vi "FuncVI-ss.vi"(5 "InstanceRef":T2, 9 "arg list":T1[](array[typedef]) {"num" format="%.2f"}) -> (0 "error out":bool, 3 "result":T1 {"num" format="%.2f"})   [LabVIEW 2021]
doc: "::: CalcExpress Toolkit :::\nCopyright (c) 2000-2026 Konstantin Shifershteyn. All rights reserved."
uses:
  cetypes.llb/CalcExpress Function Argument Info.ctl
  cetypes.llb/CalcExpress Instance RefNum.ctl
panel:
  in  "max arg num":i32=4
  in  "min arg num":i32=1
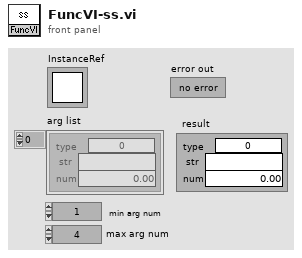
[diagram p1: front panel]
types:
  T1 = typedef "CalcExpress Function Argument Info.ctl" = cluster{"type":u32, "str":string, "num":dbl}
  T2 = typedef "CalcExpress Instance RefNum.ctl" = refnum<k1>
  T3 = cluster{"index":i32, "any type":i32, "default num":dbl, "default str":string}
  T4 = cluster{"index":i32, "data type":enum32{"String", "DBL Number", "identifier", "1D Array of DBL", "2D Array of DBL", "CDB Number", "1D Array of CDB", "2D Array of CDB", "1D Array of String", "2D Array of String", "Unknown data type"}, "default num":dbl, "default str":string}[]
  T5 = cluster{"data type":enum32{"String", "DBL Number", "identifier", "1D Array of DBL", "2D Array of DBL", "CDB Number", "1D Array of CDB", "2D Array of CDB", "1D Array of String", "2D Array of String", "Unknown data type"}, "str":string, "num":dbl}
  T6 = cluster{"index":i32, "data type":u32, "default num":dbl, "default str":string}[]
  T7 = enum32{"String", "DBL Number", "identifier", "1D Array of DBL", "2D Array of DBL", "CDB Number", "1D Array of CDB", "2D Array of CDB", "1D Array of String", "2D Array of String", "Unknown data type"}
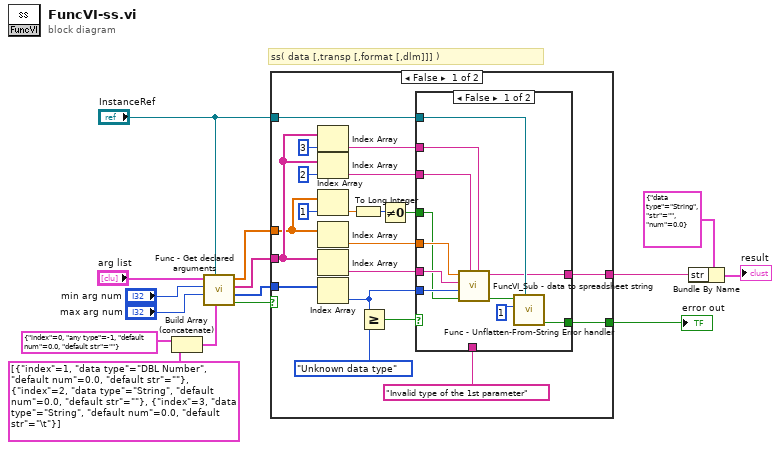
[diagram p0: block diagram]
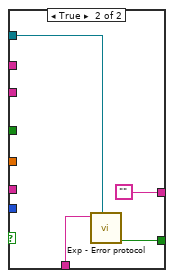
[diagram p2: hidden frame]
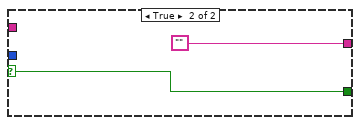
[diagram p3: hidden frame]
diagram:
  # "ss( data [,transp [,format [,dlm]]] )"
  n1 = Build Array (concatenate)(T3 {"index"=0, "any type"=-1, "default num"=0.0, "default str"=""} ("arg descriptor"), T4 [{"index"=1, "data type"=enum."DBL Number", "default num"=0.0, "default str"=""}, {"index"=2, "data type"=enum."String", "default num"=0.0, "default str"=""}, {"index"=3, "data type"=enum."String", "default num"=0.0, "default str"="\t"}] ("args descriptors")) -> (w10:T6)
  n2 = call "Func - Get declared arguments.vi"("arg descriptors"=w10, "InstanceRef"="InstanceRef", "max arg num"="max arg num", "min arg num"="min arg num", "arg list"="arg list") -> ("error out"=w9:bool, "type list"=w8:u32[], "str list"=w7:string[], "num list"=w6:dbl[])  [unwired: 3 in]
  n3 = case shown="False" w9 {
    selector: w9 -> [_ w52]
    tunnel: w8 -> [w33 _]
    tunnel: w7 -> [w32 _]
    tunnel: w6 -> [w19 _]
    tunnel: [w24 w52] -> w5
    tunnel: "InstanceRef" -> [w22 _]
    tunnel: [w21 ""] -> w3
    frame False {
      n4 = Index Array(array=w32, index=3) -> (element=w25:string)
      n5 = Index Array(array=w32, index=2) -> (element=w26:string)
      n6 = Index Array(array=w19, index=1) -> (element=w18:dbl)
      n7 = Index Array(array=w19) -> (element=w27:dbl)  [unwired: 1 in]
      n8 = Index Array(array=w32) -> (element=w28:string)  [unwired: 1 in]
      n9 = Index Array(array=w33) -> (element=w29:u32)  [unwired: 1 in]
      n10 = To Long Integer(number=w18) -> (32bit integer=w17:i32)
      n11 = Greater Or Equal?(x=w29, y=T7."Unknown data type" ("data type")) -> (x >= y?=w30:bool)
      n12 = Not Equal To 0?(x=w17) -> (x != 0?=w16:bool)
      n13 = case shown="False" w30 {
        tunnel: w29 -> [w46 _]
        tunnel: w28 -> [w45 _]
        tunnel: w27 -> [w44 _]
        tunnel: w26 -> [w43 _]
        tunnel: w25 -> [w42 _]
        tunnel: [w39 w50] -> w24
        tunnel: "Invalid type of the 1st parameter" ("ErrStr") -> [_ w49]
        tunnel: w22 -> [w38 w48]
        tunnel: [w37 ""] -> w21
        tunnel: w16 -> [w36 _]
        frame False {
          n14 = call "FuncVI_Sub - data to spreadsheet string.vi"("delimiter (Tab)"=w42, "format string"=w43, "transpose"=w36, "data type"=w46, "flattened data"=w45, "dbl"=w44) -> ("unflatten error"=w40:bool, "spreadsheet string"=w37:string)  [unwired: 2 in]
          n15 = call "Func - Unflatten-From-String Error handler.vi"("InstanceRef"=w38, "argument number"=1, "Unflatten Error status"=w40) -> ("error out"=w39:bool)  [unwired: 6 in]
        }
        frame True {
          n16 = call "Exp - Error protocol.vi"("InstanceRef"=w48, "error message in"=w49) -> ("error out"=w50:bool)  [unwired: 6 in, 1 out]
        }
      }
    }
    frame True {
    }
  }
  "error out" <- w5
  n17 = Bundle By Name(cluster=T5 {"data type"=enum."String", "str"="", "num"=0.0} ("opd info"), "str"=w3) -> (→"result":T5)
